vi "Read Speed.vi"(8 "error in (no error)":errorcluster, 11 "ETS_EM2090 in":refnum<class "ETS_EM2090.lvclass">) -> (0 "error out":errorcluster, 2 "Speed":i32 min=0 max=99, 3 "ETS_EM2090 out":refnum<class "ETS_EM2090.lvclass">)   [LabVIEW 2023, in "Turn Table and Mast.lvlib" / "ETS_EM2090.lvclass"]
uses:
  ETS_EM2090.lvclass
  ETS_EM2090.lvclass/ETS_EM2090.ctl
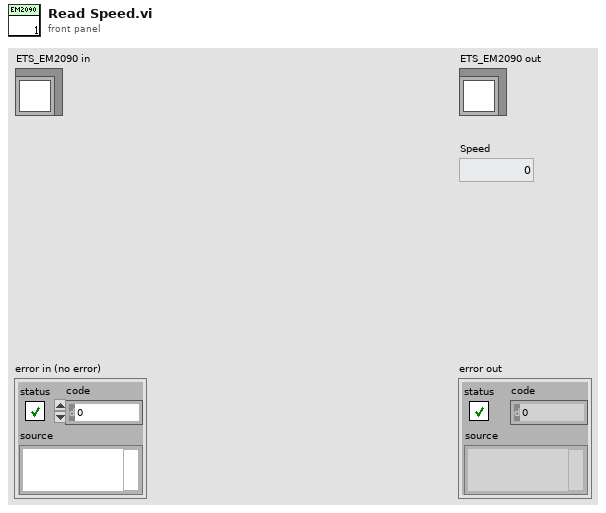
[diagram p1: front panel]
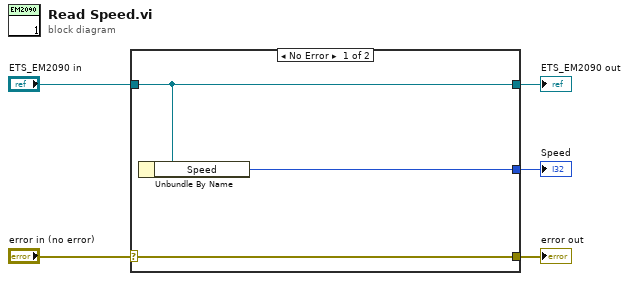
[diagram p0: block diagram]
diagram:
  n1 = case shown="No Error" "error in (no error)" {
    selector: "error in (no error)" -> [w8 w9]
    tunnel: [w8 w9] -> w4
    tunnel: [w7 w10] -> w2
    tunnel: "ETS_EM2090 in" -> [w7 w10]
    tunnel: [w6 _] -> w1
    frame No Error {
      n2 = Unbundle By Name(w7) -> ("Speed"=w6:i32)
    }
    frame Error {
    }
  }
  "error out" <- w4
  "ETS_EM2090 out" <- w2
  "Speed" <- w1
